vi "Eltochpribor RRG.vi"() -> ()   [LabVIEW 2015]
doc: "Example VI that demonstrates all library features."
uses:
  PL Eltochpribor RRG.lvclass
panel:
  in  "baudrate to set":u32(ring)=19200 items=["9600"=9600, "19200"=19200, "38400"=38400]
  in  "set address":bool
  in  "address to set":u8=1
  in  "set baudrate":bool
  in  "port":refnum<visa-resource-name>
  in  "zero":bool
  in  "flow rate, %":dbl
  out "measured flow rate, %":dbl
  in  "valve mode":u8(ring) items=["auto", "open", "closed"]
  in  "timeout, ms":u32=300
  in  "address":u8=1
  in  "baud rate":u32(ring)=19200 items=["9600"=9600, "19200"=19200, "38400"=38400]
  out "RRG":refnum<class "PL Eltochpribor RRG.lvclass">
  out "error":errorcluster
  in  "stop":bool
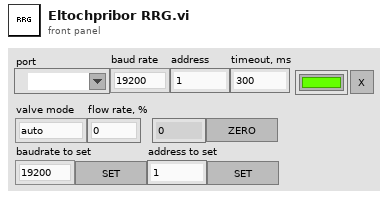
[diagram p1: front panel]
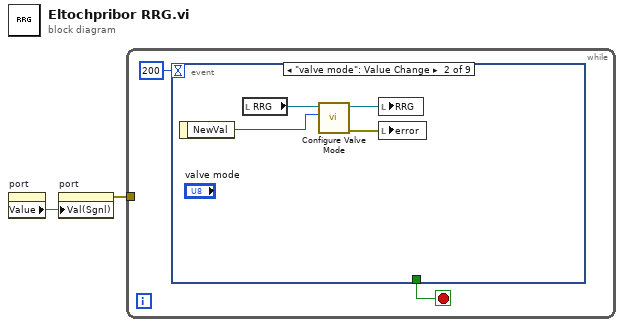
[diagram p0: block diagram]
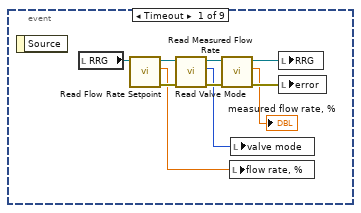
[diagram p2: hidden frame]
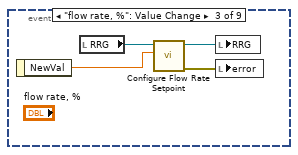
[diagram p3: hidden frame]
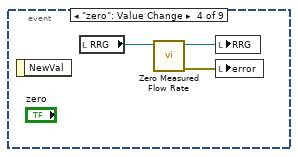
[diagram p4: hidden frame]
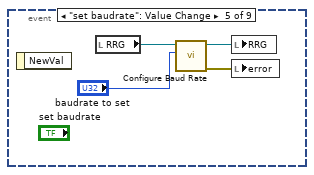
[diagram p5: hidden frame]
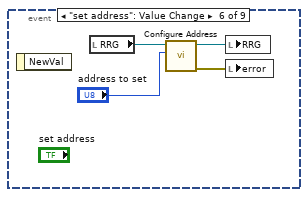
[diagram p6: hidden frame]
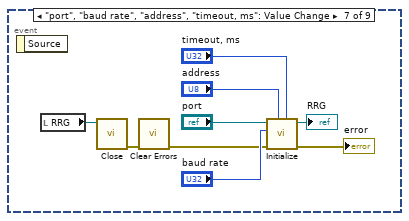
[diagram p7: hidden frame]
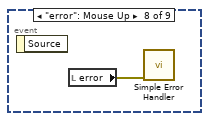
[diagram p8: hidden frame]
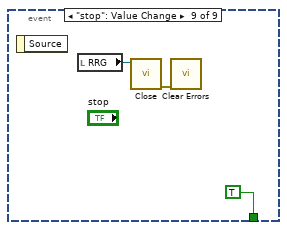
[diagram p9: hidden frame]
diagram:
  n1 = property on="port" class="VISAName"() -> ("Value"=w1:refnum<visa-resource-name>)  [unwired: 2 in, 2 out]
  n2 = property on="port" class="VISAName"("Val(Sgnl)"=w1) -> (error out=w2:errorcluster)  [unwired: 2 in, 1 out]
  n3 = while {
    tunnel: w2 -> [_]
    stop <- w3 stop-if-true
    n4 = event shown="[1] \"valve mode\": Value Change" {
      selector: _ -> [_ _ _ _ _ _ _ _ _]
      dyn-events: _ -> [_ _ _ _ _ _ _ _ _]
      timeout: 200 -> [_ _ _ _ _ _ _ _ _]
      tunnel: [_ _ _ _ _ _ _ _ TRUE ("stop")] -> w3
      event Timeout {
        n5 = event-data() -> ()  [unwired: 1 in, 1 out]
        n6 = local read "RRG"() -> (w8:refnum<class "PL Eltochpribor RRG.lvclass">)
        n7 = call "Read Flow Rate Setpoint.vi"("RRG in"=w8) -> ("error out"=w14:errorcluster, "flow rate setpoint, %"=w5:dbl, "RRG out"=w10:refnum<class "PL Eltochpribor RRG.lvclass">)  [unwired: 8 in]
        n8 = call "Read Valve Mode.vi"("error in (no error)"=w14, "RRG in"=w10) -> ("error out"=w13:errorcluster, "valve mode"=w7:u8, "RRG out"=w11:refnum<class "PL Eltochpribor RRG.lvclass">)  [unwired: 7 in]
        n9 = call "Read Measured Flow Rate.vi"("error in (no error)"=w13, "RRG in"=w11) -> ("error out"=w9:errorcluster, "measured flow rate, %"=→"measured flow rate, %":dbl, "RRG out"=w12:refnum<class "PL Eltochpribor RRG.lvclass">)  [unwired: 7 in]
        n10 = local write "flow rate, %"(w5) -> ()
        n11 = local write "valve mode"(w7) -> ()
        n12 = local write "RRG"(w12) -> ()
        n13 = local write "error"(w9) -> ()
      }
      event "valve mode": Value Change {
        n14 = event-data() -> ("NewVal"=w15:u8)  [unwired: 1 in]
        n15 = local read "RRG"() -> (w18:refnum<class "PL Eltochpribor RRG.lvclass">)
        n16 = call "Configure Valve Mode.vi"("valve mode"=w15, "RRG in"=w18) -> ("error out"=w17:errorcluster, "RRG out"=w16:refnum<class "PL Eltochpribor RRG.lvclass">)  [unwired: 8 in]
        n17 = local write "RRG"(w16) -> ()
        n18 = local write "error"(w17) -> ()
      }
      event "flow rate, %": Value Change {
        n19 = event-data() -> ("NewVal"=w19:dbl)  [unwired: 1 in]
        n20 = local read "RRG"() -> (w20:refnum<class "PL Eltochpribor RRG.lvclass">)
        n21 = call "Configure Flow Rate Setpoint.vi"("flow rate setpoint, %"=w19, "RRG in"=w20) -> ("error out"=w21:errorcluster, "RRG out"=w22:refnum<class "PL Eltochpribor RRG.lvclass">)  [unwired: 8 in]
        n22 = local write "RRG"(w22) -> ()
        n23 = local write "error"(w21) -> ()
      }
      event "zero": Value Change {
        n24 = event-data() -> ()  [unwired: 1 in, 1 out]
        n25 = local read "RRG"() -> (w24:refnum<class "PL Eltochpribor RRG.lvclass">)
        n26 = call "Zero Measured Flow Rate.vi"("RRG in"=w24) -> ("error out"=w25:errorcluster, "RRG out"=w23:refnum<class "PL Eltochpribor RRG.lvclass">)  [unwired: 9 in]
        n27 = local write "RRG"(w23) -> ()
        n28 = local write "error"(w25) -> ()
      }
      event "set baudrate": Value Change {
        n29 = event-data() -> ()  [unwired: 1 in, 1 out]
        n30 = local read "RRG"() -> (w29:refnum<class "PL Eltochpribor RRG.lvclass">)
        n31 = call "Configure Baud Rate.vi"("baud rate"="baudrate to set", "RRG in"=w29) -> ("error out"=w27:errorcluster, "RRG out"=w28:refnum<class "PL Eltochpribor RRG.lvclass">)  [unwired: 8 in]
        n32 = local write "RRG"(w28) -> ()
        n33 = local write "error"(w27) -> ()
      }
      event "set address": Value Change {
        n34 = event-data() -> ()  [unwired: 1 in, 1 out]
        n35 = local read "RRG"() -> (w31:refnum<class "PL Eltochpribor RRG.lvclass">)
        n36 = call "Configure Address.vi"("address"="address to set", "RRG in"=w31) -> ("error out"=w32:errorcluster, "RRG out"=w33:refnum<class "PL Eltochpribor RRG.lvclass">)  [unwired: 8 in]
        n37 = local write "RRG"(w33) -> ()
        n38 = local write "error"(w32) -> ()
      }
      event "port", "baud rate", "address", "timeout, ms": Value Change {
        n39 = event-data() -> ()  [unwired: 1 in, 1 out]
        n40 = local read "RRG"() -> (w37:refnum<class "PL Eltochpribor RRG.lvclass">)
        n41 = call-dynamic "Close.vi"("RRG in"=w37) -> ("error out"=w36:errorcluster)  [unwired: 10 in]
        n42 = call <vilib>:"Clear Errors.vi"("error in (no error)"=w36) -> ("error out"=w35:errorcluster)  [unwired: 5 in, 1 out]
        n43 = call "Initialize.vi"("timeout, ms (300)"="timeout, ms", "address (1)"="address", "error in (no error)"=w35, "baud rate (19200)"="baud rate", "port"="port") -> ("error out"=→"error":errorcluster, "RRG out"=→"RRG":refnum<class "PL Eltochpribor RRG.lvclass">)  [unwired: 5 in]
      }
      event "error": Mouse Up {
        n44 = event-data() -> ()  [unwired: 1 in, 1 out]
        n45 = local read "error"() -> (w43:errorcluster)
        n46 = call <vilib>:"Simple Error Handler.vi"("error in (no error)"=w43) -> ()  [unwired: 4 in, 5 out]
      }
      event "stop": Value Change {
        n47 = event-data() -> ()  [unwired: 1 in, 1 out]
        n48 = local read "RRG"() -> (w46:refnum<class "PL Eltochpribor RRG.lvclass">)
        n49 = call-dynamic "Close.vi"("RRG in"=w46) -> ("error out"=w44:errorcluster)  [unwired: 10 in]
        n50 = call <vilib>:"Clear Errors.vi"("error in (no error)"=w44) -> ()  [unwired: 5 in, 2 out]
      }
    }
  }
